vi "Test_URI_Class.vi"(8 "error in (no error)":errorcluster) -> (0 "error out":errorcluster)   [LabVIEW 2013]
uses:
  source/uri/URI.lvclass/URI.ctl
  source/components/path/URI-Component.Path.lvclass/URI-Component.Path.ctl
  source/components/query/URI-Component.Query.lvclass/URI-Component.Query.ctl
  source/uri/Read path.vi
  source/uri/Read path segments.vi
  source/uri/Read scheme.vi
  source/uri/Read username.vi
  source/uri/Read password.vi
  source/uri/Read host.vi
  source/uri/Read port.vi
  source/uri/Read Query.vi
  source/uri/Read fragment.vi
  source/utilities/Percent-Encode String.vi
  source/components/path/Get Segments.vi
  source/components/query/Get Key-Value Pairs.vi
  source/utilities/isHEXDigit.vi
  <vilib>/addons/_JKI Toolkits/Caraya/classes/Assert/Assert Equal Value_Variant.vi
  <vilib>/addons/_JKI Toolkits/Caraya/classes/Assert/Assert Equal Value and Type_Variant.vi
  source/components/path/Get path (absolute).vi
  <vilib>/Utility/error.llb/Trim Whitespace.vi
  <vilib>/addons/_JKI Toolkits/Caraya/classes/Test/Test.lvclass
  <vilib>/addons/_JKI Toolkits/Caraya/classes/Assert/Assert.lvclass
  source/uri/URI.lvclass
  source/openURI.lvlib
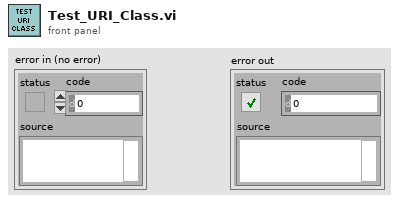
[diagram p1: front panel]
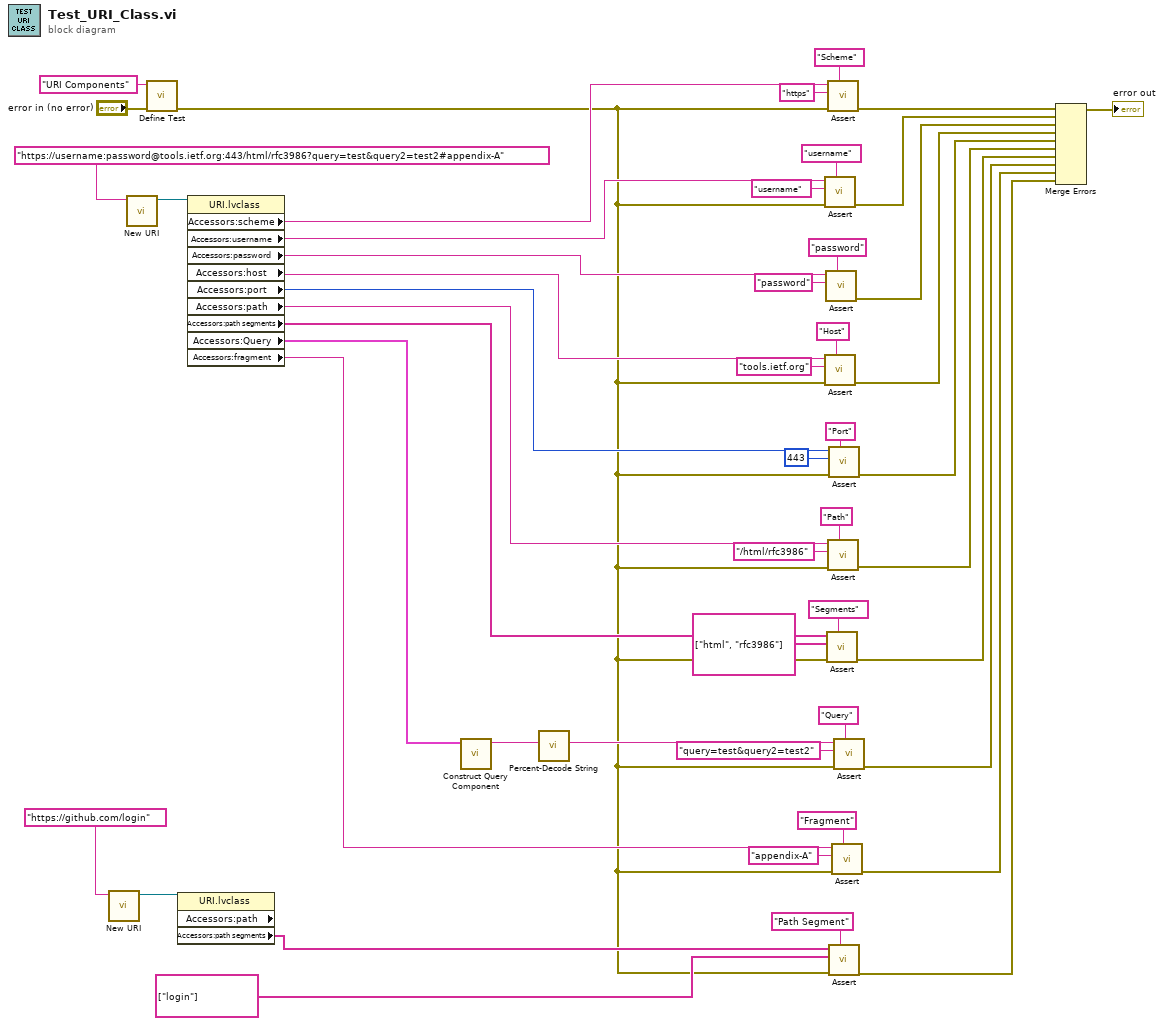
[diagram p0: block diagram]
diagram:
  n1 = call "New URI.vi"("URI"="https://github.com/login") -> ("URI"=w6:refnum<class "URI.lvclass">)  [unwired: 9 in, 1 out]
  n2 = call "New URI.vi"("URI"="https://username:password@tools.ietf.org:443/html/rfc3986?query=test&query2=test2#appendix-A") -> ("URI"=w45:refnum<class "URI.lvclass">)  [unwired: 9 in, 1 out]
  n3 = call <vilib>:"Define Test.vi"("error in (no error)"="error in (no error)", "Label (VI Title)"="URI Components") -> ("error out"=w2:errorcluster)  [unwired: 8 in, 1 out]
  n4 = property on="Property Node" class="URI.lvclass" props=["Accessors:path", "Accessors:path segments"](reference=w6) -> ("Accessors:path segments"=w3:string[])  [unwired: 1 in, 3 out]
  n5 = property on="Property Node" class="URI.lvclass"(reference=w45) -> ("Accessors:scheme"=w44:string, "Accessors:username"=w35:string, "Accessors:password"=w30:string, "Accessors:host"=w40:string, "Accessors:port"=w28:u16, "Accessors:path"=w22:string, "Accessors:path segments"=w8:string[], "Accessors:Query"=w14:cluster{"argument":string, "value":string}[], "Accessors:fragment"=w16:string)  [unwired: 1 in, 2 out]
  n6 = call "Construct Query Component.vi"("Query"=w14) -> ("query"=w10:string)  [unwired: 10 in]
  n7 = call "Percent-Decode String.vi"("Pct-Encoded String"=w10) -> ("String"=w9:string)  [unwired: 10 in]
  n8 = call-poly <vilib>:"Assert.vi"("Label"="username" ("URI"), "error in (no error)"=w2, "Y"="username" ("URI"), "X"=w35) -> ("error out"=w34:errorcluster)  [unwired: 6 in, 1 out]
  n9 = call-poly <vilib>:"Assert.vi"("Label"="Host" ("URI"), "error in (no error)"=w2, "Y"="tools.ietf.org" ("URI"), "X"=w40) -> ("error out"=w38:errorcluster)  [unwired: 6 in, 1 out]
  n10 = call-poly <vilib>:"Assert.vi"("Label"="password" ("URI"), "Y"="password" ("URI"), "X"=w30) -> ("error out"=w31:errorcluster)  [unwired: 7 in, 1 out]
  n11 = call-poly <vilib>:"Assert.vi"("Label"="Segments" ("URI"), "error in (no error)"=w2, "Y"=string[] ["html", "rfc3986"] ("Segments"), "X"=w8) -> ("error out"=w19:errorcluster)  [unwired: 6 in, 1 out]
  n12 = call-poly <vilib>:"Assert.vi"("Label"="Scheme" ("URI"), "error in (no error)"=w2, "Y"="https" ("URI"), "X"=w44) -> ("error out"=w39:errorcluster)  [unwired: 6 in, 1 out]
  n13 = call-poly <vilib>:"Assert.vi"("Label"="Path" ("URI"), "error in (no error)"=w2, "Y"="/html/rfc3986" ("URI"), "X"=w22) -> ("error out"=w23:errorcluster)  [unwired: 6 in, 1 out]
  n14 = call-poly <vilib>:"Assert.vi"("Label"="Port" ("URI"), "error in (no error)"=w2, "Y"=u16 443 ("port"), "X"=w28) -> ("error out"=w26:errorcluster)  [unwired: 6 in, 1 out]
  n15 = call-poly <vilib>:"Assert.vi"("Label"="Path Segment" ("URI"), "error in (no error)"=w2, "Y"=string[] ["login"] ("Segments"), "X"=w3) -> ("error out"=w1:errorcluster)  [unwired: 6 in, 1 out]
  n16 = call-poly <vilib>:"Assert.vi"("Label"="Fragment" ("URI"), "error in (no error)"=w2, "Y"="appendix-A" ("URI"), "X"=w16) -> ("error out"=w15:errorcluster)  [unwired: 6 in, 1 out]
  n17 = call-poly <vilib>:"Assert.vi"("Label"="Query" ("URI"), "error in (no error)"=w2, "Y"="query=test&query2=test2" ("URI"), "X"=w9) -> ("error out"=w11:errorcluster)  [unwired: 6 in, 1 out]
  n18 = Merge Errors(w39, w34, w31, w38, w26, w23, w19, w11, w15, w1) -> (→"error out":errorcluster)
